vi "UtilityOp Default.vi"(10 "Occurrence Refnum":refnum<k4>, 11 "OpMode Index":u64 format="%.0x") -> ()   [LabVIEW 2023]
uses:
  <vilib>/MRC/MrcLib.lvlib
  <vilib>/MRC/Types/WPI_JoystickDeviceEnum.ctl
panel:
  out "RobotMode":u8
  out "Match Time(s)":sgl
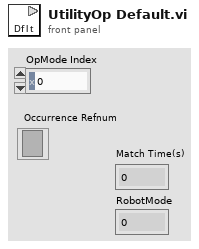
[diagram p1: front panel]
types:
  T1 = typedef "WPI_JoystickDeviceEnum.ctl" = enum16{"USB 0", "USB 1", "USB 2", "USB 3", "USB 4", "USB 5"}
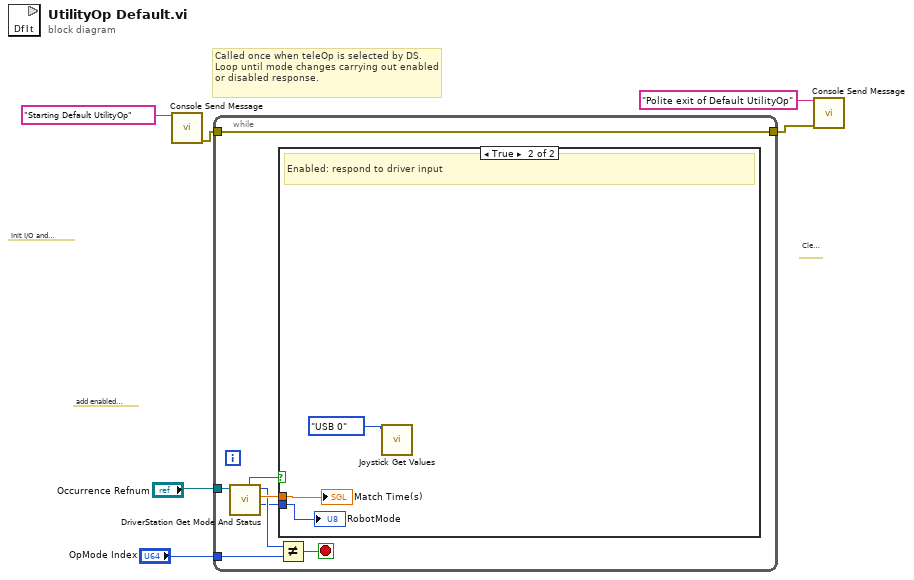
[diagram p0: block diagram]
diagram:
  # "Called once when teleOp is selected by DS.\nLoop until mode changes carrying out enabled\nor disabled response."
  # "add enabled counter\nstats, etc"
  # "Cleanup I/O"
  # "Init I/O and anything\nused during TeleOp"
  n1 = call <vilib>:"Console Send Message.vi"("Message"="Starting Default UtilityOp") -> ("error out"=w2:errorcluster)  [unwired: 14 in]
  n2 = while {
    tunnel: "OpMode Index" -> [w12]
    tunnel: [w8] -> w3
    tunnel: w2 -> [w8]
    tunnel: "Occurrence Refnum" -> [w7]
    stop <- w11 stop-if-true
    n3 = call <vilib>:"DriverStation Get Mode And Status.vi"("Occurrence Refnum"=w7) -> ("RobotMode"=w9:u8, "Match Time(s)"=w14:sgl, "currentOpMode"=w10:u64, "Enabled"=w13:bool)  [unwired: 5 in, 2 out]
    n4 = Not Equal?(x=w10, y=w12) -> (x != y?=w11:bool)
    n5 = case shown="True" w13 {
      tunnel: w14 -> [_ w17]
      tunnel: w9 -> [_ w16]
      frame False {
        # "Disabled: update dashboard, possibly update state and setpoints for safer enable"
      }
      frame True {
        # "Enabled: respond to driver input"
        n6 = call <vilib>:"Joystick Get Values.vi"("Joystick"=WPI_JoystickDeviceEnum."USB 0") -> ()  [unwired: 5 in, 6 out]
        "Match Time(s)" <- w17
        "RobotMode" <- w16
      }
    }
  }
  n7 = call <vilib>:"Console Send Message.vi"("Message"="Polite exit of Default UtilityOp", "error in (no error)"=w3) -> ()  [unwired: 13 in, 1 out]
